vi "JKI SM EDITOR - quick filter list.vi"(0 "quick filter text":string, 1 "Num Event Frames":i32, 7 "States":string[](array[string]), 11 "error in":errorcluster) -> (6 "All Items Filtered Out":bool, 8 "States quick-filtered":string[](array[string]), 10 "Indices quick-filtered":i32[](array[numeric]), 15 "error out":errorcluster)   [LabVIEW 2020]
uses:
  JKI State Machine API/source/JKI SM/JKI SM.lvclass
panel:
  # "Copyright © 2006 James Kring, Inc. All rights reserved.\nMichael Aivaliotis michael.aivaliotis@jameskring.com\nalternate email: michael@aivaliotis.com\n\nThis library is provided \"AS IS\" , WITHOUT WARRANTIES OR \nCONDITIONS OF ANY KIND, either express or implied.\n\nJames Kring, Inc. -- http://www.jameskring.com"
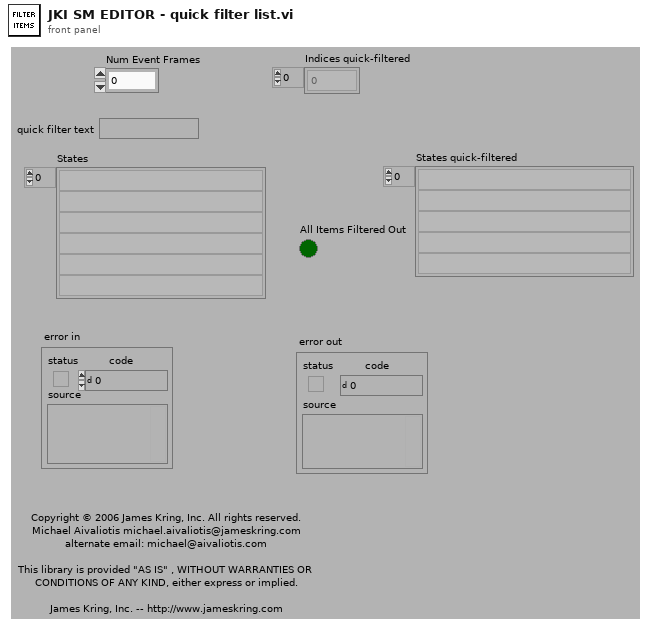
[diagram p1: front panel]
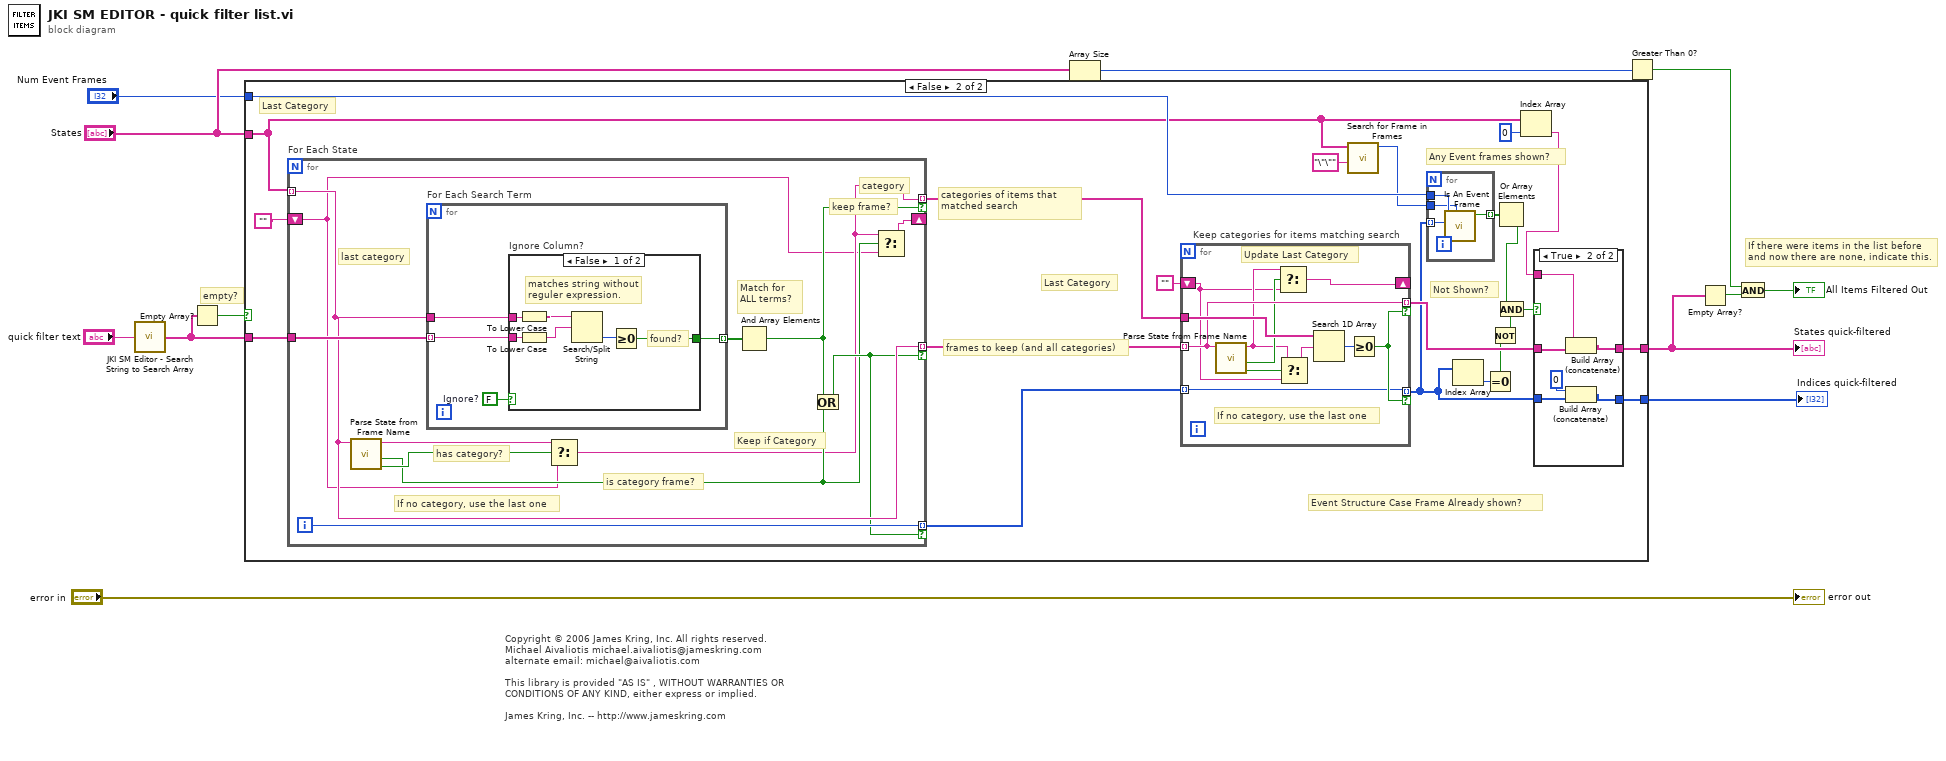
[diagram p0: block diagram]
diagram:
  # "If there were items in the list before and now there are none, indicate this."
  # "Copyright © 2006 James Kring, Inc. All rights reserved.\nMichael Aivaliotis michael.aivaliotis@jameskring.com\nalternate email: michael@aivaliotis.com\n\nThis library is provided \"AS IS\" , WITHOUT WARRANTIES OR \nCONDITIONS OF ANY KIND, either express or implied.\n\nJames Kring, Inc. -- http://www.jameskring.com"
  # "empty?"
  n1 = call "JKI SM Editor - Search String to Search Array.vi"("String"="quick filter text") -> ("Array"=w5:string[])
  n2 = Empty Array?(array=w5) -> (empty?=w4:bool)
  n3 = case shown="False" w4 {
    tunnel: w5 -> [_ w37]
    tunnel: "States" -> [w14 w17]
    tunnel: [w14 w29] -> w11
    tunnel: [w13 w28] -> w2
    tunnel: "Num Event Frames" -> [_ w33]
    frame True {
      # "return previous list untouched."
      n4 = for {
        tunnel: w14 -> [_] mode=indexing
        tunnel: [w15] -> w13 mode=indexing
        i -> [w15]
      }
    }
    frame False {
      # "Last Category"
      # "Last Category"
      # "Any Event frames shown?"
      # "Not Shown?"
      # "Event Structure Case Frame Already shown?"
      # "categories of items that matched search"
      # "frames to keep (and all categories)"
      n5 = for "For Each State" {
        tunnel: w17 -> [w69] mode=indexing
        tunnel: w37 -> [w72]
        tunnel: [w69] -> w34 mode=indexing if=w67
        tunnel: [w62] -> w36 mode=indexing if=w70
        tunnel: [w68] -> w35 mode=indexing if=w67
        shift-right: [w64] -> _
        shift-left: "" -> [w61]
        i -> [w68]
        # "last category"
        # "is category frame?"
        # "If no category, use the last one"
        # "Keep if Category"
        # "category"
        # "keep frame?"
        # "has category?"
        # "Match for ALL terms?"
        n6 = call "Parse State from Frame Name.vi"("Frame or State Name"=w69) -> ("Has Category?"=w66:bool, "is a Category Frame?"=w63:bool, "Category Name"=w65:string)  [unwired: 5 in, 3 out]
        n7 = for "For Each Search Term" {
          tunnel: w69 -> [w76]
          tunnel: w72 -> [w75] mode=indexing
          tunnel: [w74] -> w71 mode=indexing
          w73 = FALSE  # Ignore?
          n8 = case "Ignore Column?" shown="False" w73 {
            tunnel: w76 -> [w82 _]
            tunnel: w75 -> [w81 _]
            tunnel: [w77 _] -> w74
            frame False {
              # "matches string without reguler expression."
              # "found?"
              n9 = To Lower Case(string=w82) -> (all lower case string=w80:string)
              n10 = To Lower Case(string=w81) -> (all lower case string=w79:string)
              n11 = Search/Split String(string=w80, search string/char (-)=w79) -> (offset of match=w78:i32)  [unwired: 1 in, 2 out]
              n12 = Greater Or Equal To 0?(x=w78) -> (x >= 0?=w77:bool)
            }
            frame True {
            }
          }
        }
        n13 = Select(t=w65, s=w66, f=w61) -> (s? t:f=w62:string)
        n14 = And Array Elements(Boolean array=w71) -> (logical AND=w70:bool)
        n15 = Or(x=w70, y=w63) -> (x .or. y?=w67:bool)
        n16 = Select(t=w62, s=w63, f=w61) -> (s? t:f=w64:string)
      }
      n17 = for "Keep categories for items matching search" {
        tunnel: w34 -> [w59] mode=indexing
        tunnel: w36 -> [w60]
        tunnel: [w59] -> w30 mode=indexing if=w57
        tunnel: [w56] -> w26 mode=indexing if=w57
        tunnel: w35 -> [w56] mode=indexing
        shift-right: [w54] -> _
        shift-left: "" -> [w50]
        # "If no category, use the last one"
        # "Update Last Category"
        n18 = call "Parse State from Frame Name.vi"("Frame or State Name"=w59) -> ("Has Category?"=w53:bool, "is a Category Frame?"=w55:bool, "Category Name"=w52:string)  [unwired: 5 in, 3 out]
        n19 = Select(t=w52, s=w55, f=w50) -> (s? t:f=w54:string)
        n20 = Select(t=w52, s=w53, f=w50) -> (s? t:f=w51:string)
        n21 = Search 1D Array(1D array=w60, element=w51) -> (index of element=w58:i32)  [unwired: 1 in]
        n22 = Greater Or Equal To 0?(x=w58) -> (x >= 0?=w57:bool)
      }
      n23 = call "Search for Frame in Frames.vi"("Frame Name"="\"\"", "Frame Names"=w17) -> ("index of element"=w16:i32)  [unwired: 9 in]
      n24 = for {
        tunnel: w26 -> [w49] mode=indexing
        tunnel: w33 -> [w48]
        tunnel: [w47] -> w32 mode=indexing
        tunnel: w16 -> [w46]
        n25 = call "Is An Event Frame.vi"("Event Structure index"=w46, "index of element"=w49, "Num Event Frames"=w48) -> ("Event Frame?"=w47:bool)  [unwired: 7 in, 1 out]
      }
      n26 = Index Array(array=w26) -> (element=w25:i32)  [unwired: 1 in]
      n27 = Equal To 0?(x=w25) -> (x = 0?=w24:bool)
      n28 = Not(x=w24) -> (.not. x?=w21:bool)
      n29 = Or Array Elements(Boolean array=w32) -> (logical OR=w23:bool)
      n30 = And(x=w23, y=w21) -> (x .and. y?=w22:bool)
      n31 = Index Array(array=w17, index=0) -> (element=w27:string)
      n32 = case shown="True" w22 {
        tunnel: [w39 w43] -> w29
        tunnel: w30 -> [w39 w44]
        tunnel: [w38 w41] -> w28
        tunnel: w26 -> [w38 w42]
        tunnel: w27 -> [_ w45]
        frame False {
        }
        frame True {
          n33 = Build Array (concatenate)(w45, w44) -> (w43:string[])
          n34 = Build Array (concatenate)(0 ("index"), w42) -> (w41:i32[])
        }
      }
    }
  }
  "States quick-filtered" <- w11
  "Indices quick-filtered" <- w2
  n35 = Array Size(array="States") -> (size(s)=w7:i32)
  n36 = Greater Than 0?(x=w7) -> (x > 0?=w8:bool)
  n37 = Empty Array?(array=w11) -> (empty?=w10:bool)
  n38 = And(x=w8, y=w10) -> (x .and. y?=→"All Items Filtered Out":bool)
  "error out" <- "error in"
